vi "FlatSequenceToJson.vi"(6 "Current Path":path, 7 "Origin Path":path, 8 "error in":errorcluster, 9 "Component Idx":i32, 10 "Relative Bounds":cluster{"x":i32, "y":i32, "w":i32, "h":i32}, 11 "FlatSequence in":refnum<vi>) -> (0 "error out":errorcluster, 3 "JSON":string)   [LabVIEW 2017]
doc: "Converts a flat sequence structure into a JSON"
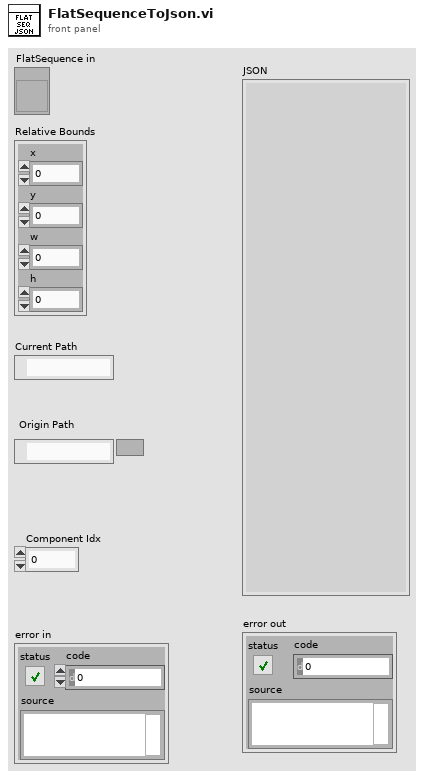
[diagram p1: front panel]
types:
  T1 = typedef "LVRectTypeDef.ctl" = cluster{"Left":i16, "Top":i16, "Right":i16, "Bottom":i16}
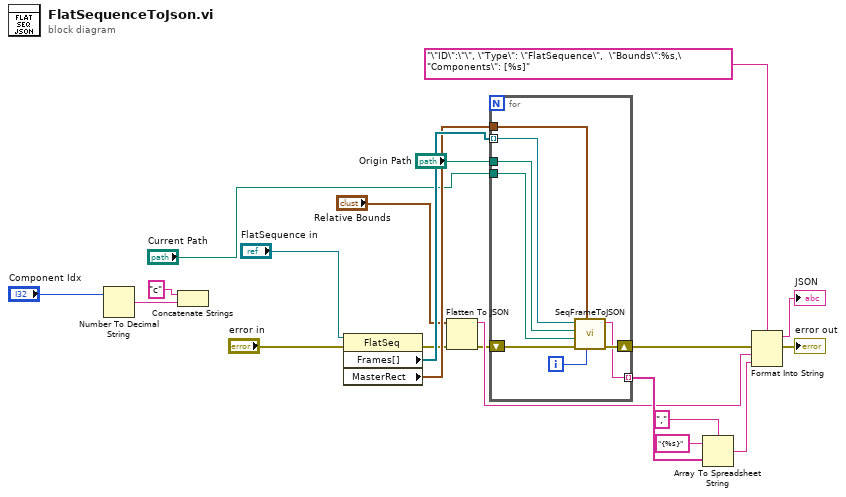
[diagram p0: block diagram]
diagram:
  n1 = Number To Decimal String(number="Component Idx") -> (decimal integer string=w12:string)  [unwired: 1 in]
  n2 = Concatenate Strings("c" ("string"), w12) -> ()  [unwired: 1 out]
  n3 = property class="FlatSeq"(reference="FlatSequence in", error in="error in") -> (error out=w3:errorcluster, "Frames[]"=w20:refnum<vi>[], "MasterRect"=w15:T1)  [unwired: 1 out]
  n4 = Flatten To JSON(anything="Relative Bounds", error in (no error)=w3) -> (JSON string=w4:string, 11:w2:errorcluster)  [unwired: 1 in]
  n5 = for {
    tunnel: w20 -> [w29] mode=indexing
    shift-right: [w23] -> w18
    shift-left: w2 -> [w25]
    tunnel: w15 -> [w28]
    tunnel: "Current Path" -> [w27]
    tunnel: "Origin Path" -> [w24]
    tunnel: [w22] -> w9 mode=indexing
    i -> [w26]
    n6 = call "SeqFrameToJSON.vi"("Numeric"=w26, "MasterRect"=w28, "error in (no error)"=w25, "created path"=w27, "Origin Path"=w24, "FlatSequenceFrame in"=w29) -> ("error out"=w23:errorcluster, "JSON"=w22:string)  [unwired: 4 in]
  }
  n7 = Array To Spreadsheet String(delimiter (Tab)=",", array=w9, 3:"{%s}" ("format string")) -> (spreadsheet string=w6:string)
  n8 = Format Into String(format string="\"ID\":\"\", \"Type\": \"FlatSequence\",  \"Bounds\":%s,\"Components\": [%s]", error in=w18, w4, w6) -> (resulting string=→"JSON":string, error out=→"error out":errorcluster)  [unwired: 1 in]
